vi "hp8903b 生成xy图像（低频）.vi"(3 "error in (no error)":errorcluster, 4 "detector selection\n(no change)":u16(ring) items=["no change", "rms", "average", "quasi-peak"], 5 "measurements\n(AC level)":u16(ring) items=["AC level", "DC level", "Distortion", "Distortion level", "Signal-to-Noise", "SINAD"]) -> (0 "error out":errorcluster, 1 "value read":dbl format="%.7f")   [LabVIEW 2023]
doc: "This vi uses several of the lower level vi's to configure the audio analyzer and take a measurement. It also initializes, resets, and then finally closes the instrument."
panel:
  out "Waveform Chart":dbl[](graph)
  in  "stop":bool
  in  "VISA resource name":refnum<visa-resource-name>
  in  "SINAD meter range\n(f:0 to 18)":bool
  in  "range selector\n(f:except DC)":bool
  in  "input level range(DC only)\n(auto select)":u16(ring) items=["automatic select", "300V", "64V", "16V", "4V"]
  in  "input level range(except DC)\n(auto select)":u16(ring) items=["automatic select", "300V", "189V", "119V", "75.4V", "47.6V", "30.0V", "18.9V", "11.9V", "7.54V", "4.76V", "3.00V", "1.89V", "1.19V", "0.754V", "0.476V", "0.300V", "0.189V", "0.119V", "0.0754V"]
  in  "set reference value\n(no:f)":bool
  in  "reference value (0)":dbl format="%.5f"
  in  "measurement mode\n(LIN:f)":bool
  # "configure measurements"
  # "LOG"
  # "range configurations"
  # "LIN"
  # "yes"
  # "no"
  # "0 to 24 dB"
  # "0 to 18 dB"
  # "input range (DC only)"
  # "input range (except DC)"
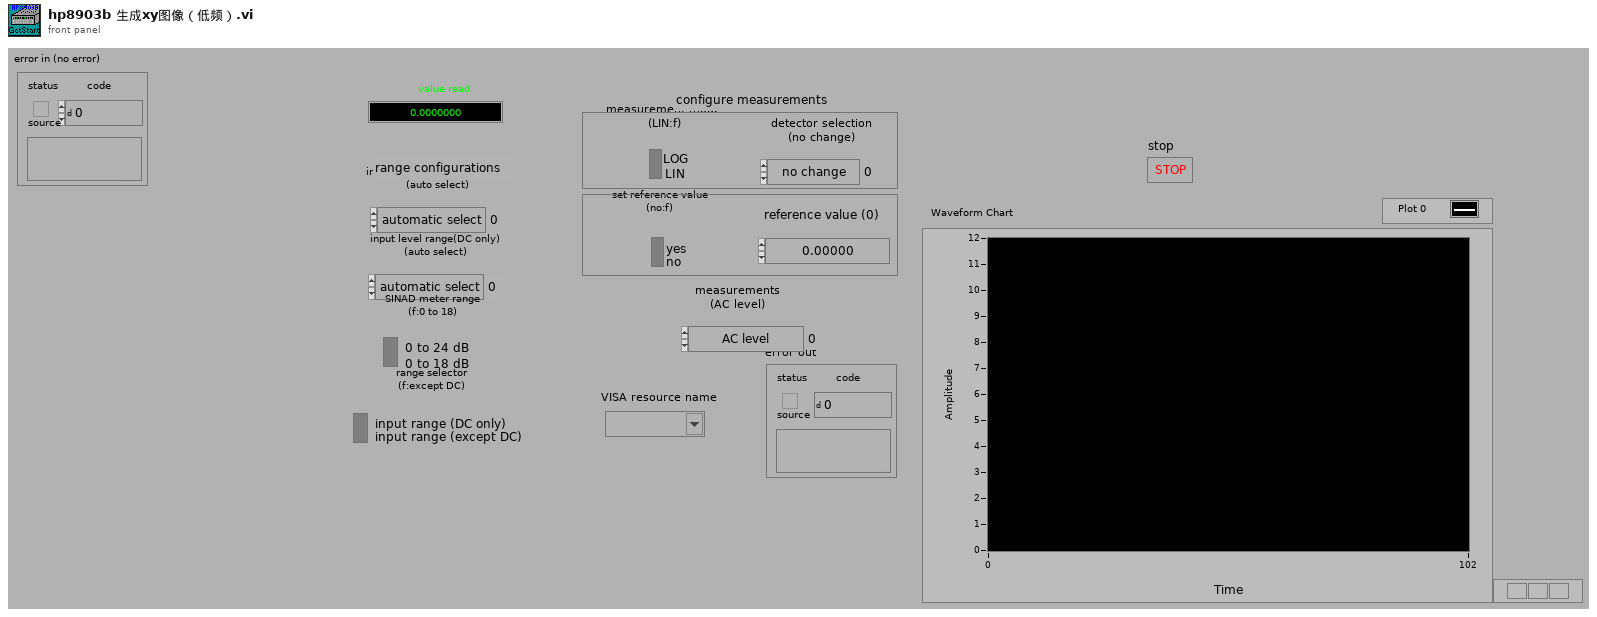
[diagram p1: front panel]
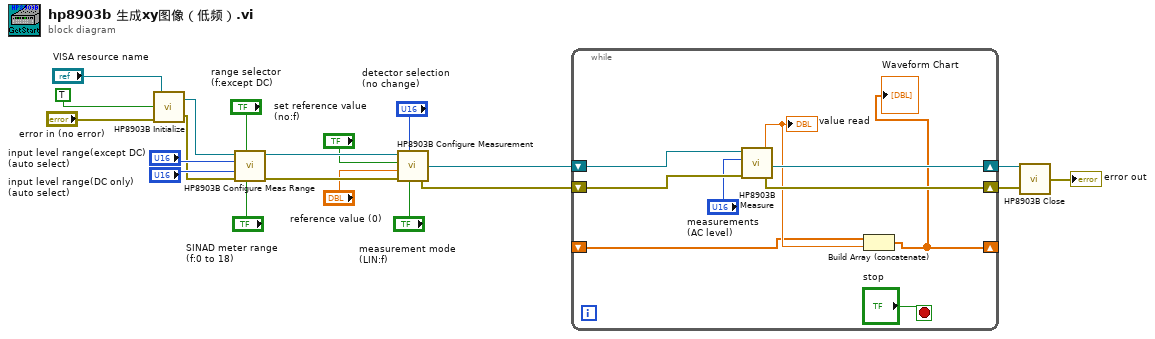
[diagram p0: block diagram]
diagram:
  n1 = call <instrlib>:"HP8903B Initialize.vi"("error in (no error)"="error in (no error)", "reset (no : F)"=TRUE, "VISA resource name"="VISA resource name") -> ("error out"=w6:errorcluster, "VISA session"=w8:refnum<visa-resource-name>)  [unwired: 1 in]
  n2 = call <instrlib>:"HP8903B Configure Meas Range.vi"("SINAD meter range\n(f:0 to 18)"="SINAD meter range\n(f:0 to 18)", "range selector\n(f:except DC)"="range selector\n(f:except DC)", "error in (no error)"=w6, "input level range : DC only\n(auto select)"="input level range(DC only)\n(auto select)", "input level range : except DC\n(auto select)"="input level range(except DC)\n(auto select)", "VISA session"=w8) -> ("error out"=w16:errorcluster, "dup VISA session"=w15:refnum<visa-resource-name>)
  n3 = call <instrlib>:"HP8903B Configure Measurement.vi"("measurement mode\n(LIN:f)"="measurement mode\n(LIN:f)", "detector selection\n(no change)"="detector selection\n(no change)", "error in (no error)"=w16, "reference value (0)"="reference value (0)", "set reference value\n(no:f)"="set reference value\n(no:f)", "VISA session"=w15) -> ("error out"=w10:errorcluster, "dup VISA session"=w9:refnum<visa-resource-name>)
  n4 = while {
    shift-right: [w25] -> w3
    shift-left: w10 -> [w29]
    shift-right: [w26] -> w4
    shift-left: w9 -> [w28]
    shift-right: [w21] -> _
    shift-left: _ -> [w22]
    stop <- "stop" stop-if-true
    n5 = call <instrlib>:"HP8903B Measure.vi"("error in (no error)"=w29, "measurements\n(AC level)"="measurements\n(AC level)", "VISA session"=w28) -> ("error out"=w25:errorcluster, "value read"=w23:dbl, "dup VISA session"=w26:refnum<visa-resource-name>)  [unwired: 1 in]
    "value read" <- w23
    n6 = Build Array (concatenate)(w22, w23) -> (w21:dbl[])
    "Waveform Chart" <- w21
  }
  n7 = call <instrlib>:"HP8903B Close.vi"("error in (no error)"=w3, "VISA session"=w4) -> ("error out"=→"error out":errorcluster)
